vi "ValueSignalByPathString.vi"(0 "VI Reference In":refnum<vi>, 2 "delimiter (>>)":string=">>", 5 "Control Path":string, 7 "Value (Signaling)":variant, 11 "error in":errorcluster) -> (4 "VI Reference Out":refnum<vi>, 15 "error out":errorcluster)   [LabVIEW 2016, in "Drona.lvlib" / "ControlValue.lvlib"]
doc: "Sets value(signaling) for the control which is specified. \n\nThe input control name is given as a string , incase of path, use delimiters inbetween the path."
uses:
  ControlValue.lvlib
  Drona.lvlib
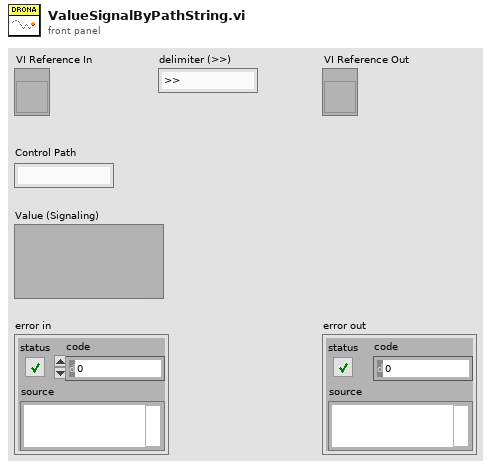
[diagram p1: front panel]
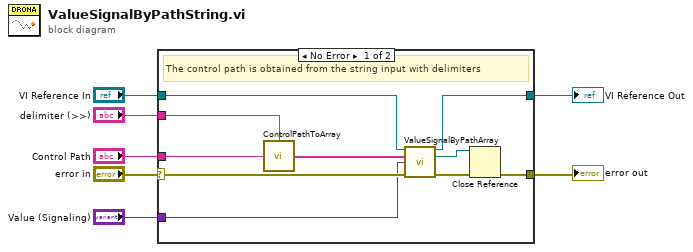
[diagram p0: block diagram]
diagram:
  n1 = case shown="No Error" "error in" {
    selector: "error in" -> [w17 w19]
    tunnel: "Control Path" -> [w13 _]
    tunnel: "VI Reference In" -> [w15 w18]
    tunnel: [w14 w18] -> w4
    tunnel: "Value (Signaling)" -> [w16 _]
    tunnel: [w8 w19] -> w2
    tunnel: "delimiter (>>)" -> [w11 _]
    frame No Error {
      # "The control path is obtained from the string input with delimiters"
      n2 = call "ControlPathToArray.vi"("Control Name"=w13, "delimiter (>>)"=w11) -> ("Control Path"=w12:string[])
      n3 = call "ValueSignalByPathArray.vi"("VI Reference In"=w15, "Control Path"=w12, "Value (Signaling)"=w16, "Error In"=w17) -> ("VI Reference Out"=w14:refnum<vi>, "Ctl Reference Out"=w9:refnum<vi>, "Error Out"=w10:errorcluster)  [unwired: 9 in]
      n4 = Close Reference(reference=w9, error in (no error)=w10) -> (error out=w8:errorcluster)
    }
    frame Error {
    }
  }
  "error out" <- w2
  "VI Reference Out" <- w4
